vi "Spreading.vi"() -> ()   [LabVIEW 2023]
panel:
  out "Spread Output":i16[](array[numeric])
  in  "PRN Chips":i16[](array[numeric])
  in  "GPS Word (U32)":u32
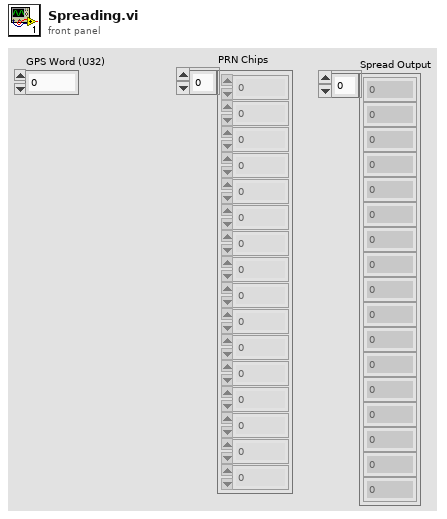
[diagram p1: front panel]
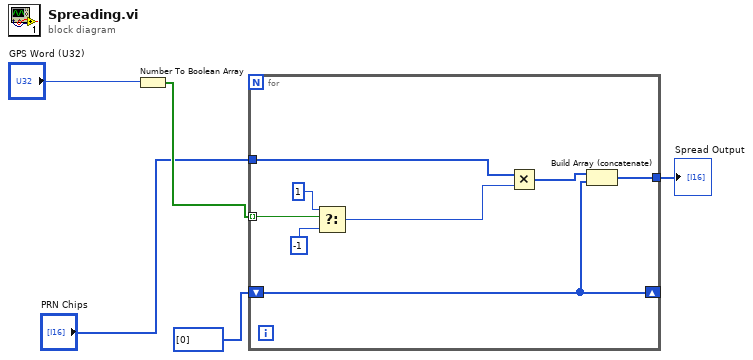
[diagram p0: block diagram]
diagram:
  n1 = Number To Boolean Array(number="GPS Word (U32)") -> (Boolean array=w4:bool[])
  n2 = for {
    tunnel: w4 -> [w13] mode=indexing
    tunnel: "PRN Chips" -> [w9]
    shift-right: [w7] -> _
    shift-left: i16[] [0] -> [w7]
    tunnel: [w6] -> w1
    n3 = Select(t=i16 1, s=w13, f=i16 -1) -> (s? t:f=w10:i16)
    n4 = Multiply(x=w9, y=w10) -> (x*y=w8:i16[])
    n5 = Build Array (concatenate)(w8, w7) -> (w6:i16[])
  }
  "Spread Output" <- w1
